vi "user process.vi"(8 "error in":errorcluster, 10 "ExampleStateMachine runtime in":refnum<class "ExampleStateMachine runtime.lvclass">, 11 "Parameters to process":T3) -> (0 "error out":errorcluster, 2 "ExampleStateMachine runtime out":refnum<class "ExampleStateMachine runtime.lvclass">, 3 "Results from processing":T2)   [LabVIEW 2017, in "ExampleStateMachine runtime.lvclass"]
uses:
  ExampleStateMachine runtime.lvclass
  parameter user data.ctl
  result user data.ctl
  Utilities/StateMachine.ctl
  Utilities/Controlword_Commands.ctl
  CommandCluster.ctl
  Utilities/WordManipulationLibrary.lvlib
panel:
  out "Status":T1
  out "Results":dbl[](array[numeric])
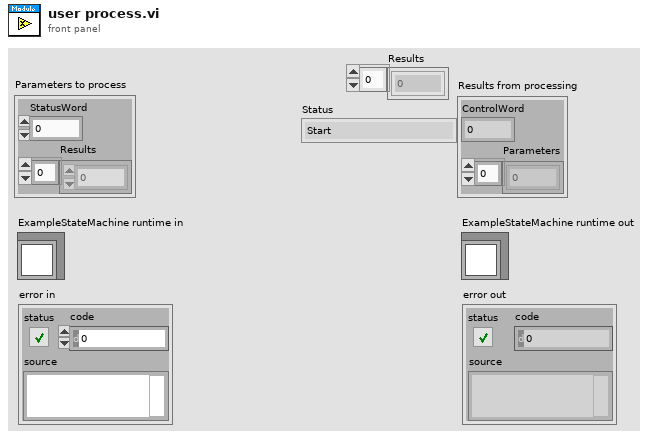
[diagram p1: front panel]
types:
  T1 = typedef "WordManipulationLibrary.lvlib/StateMachine.ctl" = enum16{"Start", "Not Ready to Switch On", "Switch On Disabled", "Ready to Switch On", "Switched On", "Operation enable", "Quick Stop Active", "Fault Reaction Active", "Fault"}
  T2 = typedef "ExampleStateMachine runtime.lvclass/result user data.ctl" = cluster{"ControlWord":u16, "Parameters":dbl[]}
  T3 = typedef "ExampleStateMachine runtime.lvclass/parameter user data.ctl" = cluster{"StatusWord":u16, "Results":dbl[]}
  T4 = typedef "WordManipulationLibrary.lvlib/Controlword_Commands.ctl" = enum16{"Shutdown", "Switch On", "Disable Voltage", "Quick Stop", "Disable Op", "Enable Op", "Fault Reset", "Error"}
  T5 = enum16{"Shutdown", "Switch On", "Disable Voltage", "Quick Stop", "Disable Op", "Enable Op", "Fault Reset", "Error"}
  T6 = typedef "CommandCluster.ctl" = cluster{"Modes":enum16{"Reserved", "Profile Position Mode", "Velocity Mode", "Profile Velocity Mode", "Profile Torque Mode", "Reserved 2", "Reference Mode", "Interpolated Position Mode", "Skip"}, "Parameters_PositionProfile":dbl[]}
  T7 = enum16{"Reserved", "Profile Position Mode", "Velocity Mode", "Profile Velocity Mode", "Profile Torque Mode", "Reserved 2", "Reference Mode", "Interpolated Position Mode", "Skip"}
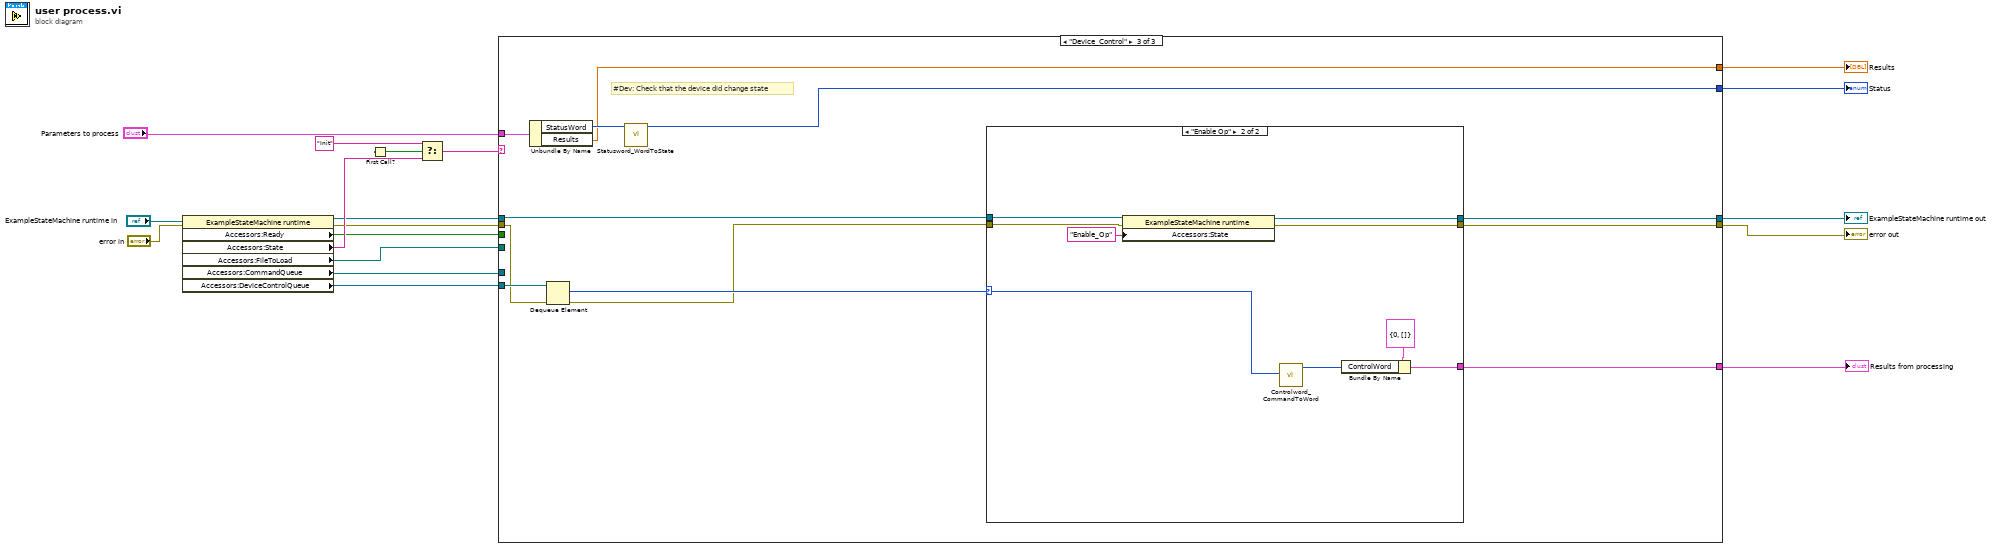
[diagram p0: block diagram]
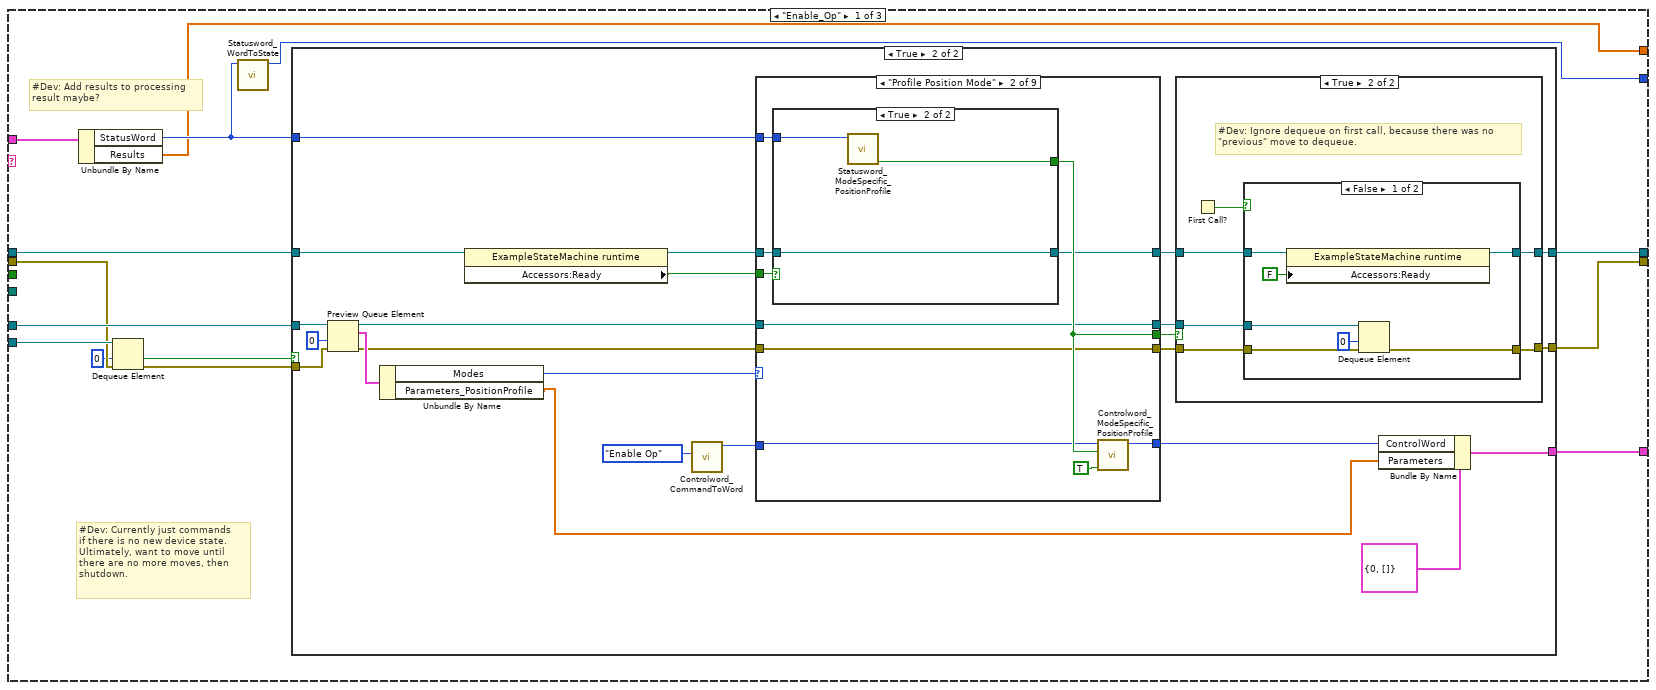
[diagram p2: hidden frame]
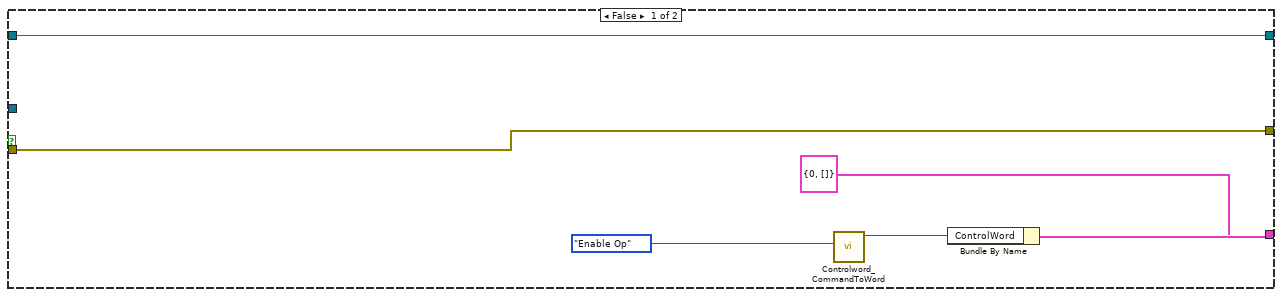
[diagram p3: hidden frame]
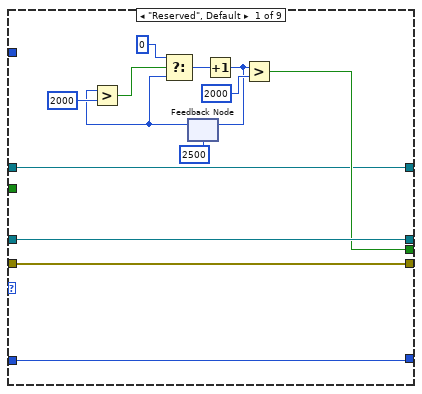
[diagram p6: hidden frame]
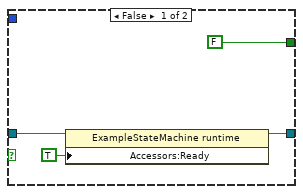
[diagram p7: hidden frame]
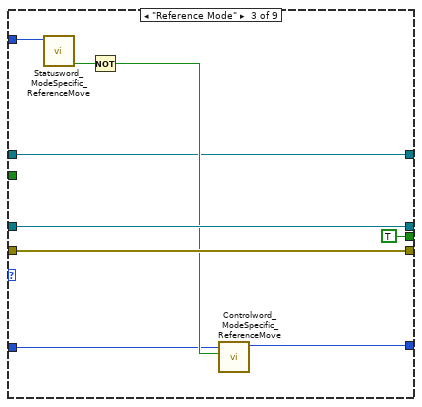
[diagram p8: hidden frame]
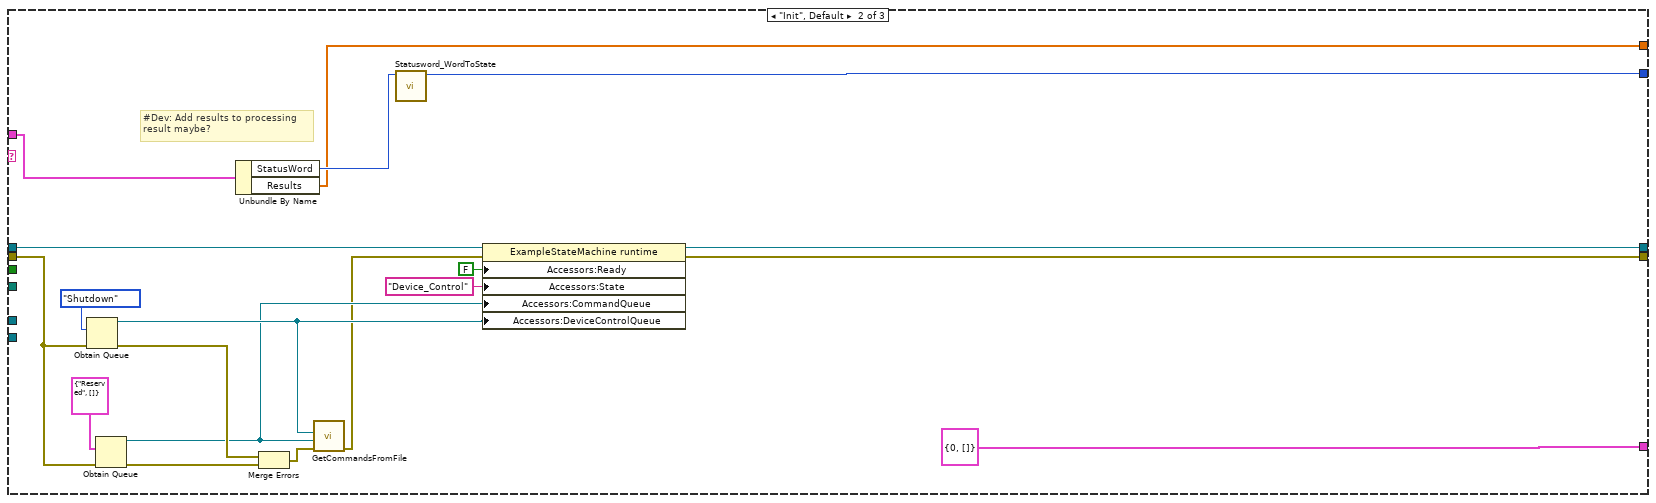
[diagram p15: hidden frame]
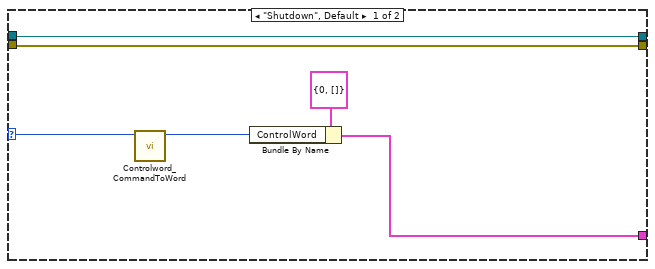
[diagram p16: hidden frame]
diagram:
  n1 = property class="ExampleStateMachine runtime"(reference="ExampleStateMachine runtime in", error in="error in") -> (reference out=w9:refnum<class "ExampleStateMachine runtime.lvclass">, error out=w7:errorcluster, "Accessors:Ready"=w5:bool, "Accessors:State"=w16:string, "Accessors:FileToLoad"=w10:path, "Accessors:CommandQueue"=w3:refnum<queue>, "Accessors:DeviceControlQueue"=w4:refnum<queue>)
  n2 = First Call?() -> (First Call?: T/F=w18:bool)
  n3 = Select(t="Init" ("f"), s=w18, f=w16) -> (s? t:f=w13:string)
  n4 = case shown="\"Device_Control\"" w13 {
    tunnel: "Parameters to process" -> [w26 w144 w170]
    tunnel: [w27 T2 {"ControlWord"=0, "Parameters"=[]} ("Results from processing") w172] -> w11
    tunnel: w10 -> [_ _ _]
    tunnel: w9 -> [w31 w159 w171]
    tunnel: [w24 w158 w166] -> w8
    tunnel: w7 -> [w29 w155 w165]
    tunnel: [w25 w157 w163] -> w6
    tunnel: w5 -> [_ _ _]
    tunnel: w4 -> [w32 _ w168]
    tunnel: w3 -> [w30 _ _]
    tunnel: [w22 w143 w162] -> w2
    tunnel: [w21 w142 w161] -> w1
    frame "Enable_Op" {
      # "#Dev: Add results to processing\nresult maybe?"
      # "#Dev: Currently just commands\nif there is no new device state.\nUltimately, want to move until\nthere are no more moves, then\nshutdown."
      n5 = Unbundle By Name(w26) -> ("StatusWord"=w23:u16, "Results"=w21:dbl[])
      n6 = Dequeue Element(queue=w32, timeout in ms (-1)=0, error in (no error)=w29) -> (timed out?=w19:bool, error out=w28:errorcluster)  [unwired: 2 out]
      n7 = call "Statusword_WordToState.vi"("Data_In"=w23) -> ("Status"=w22:T1)  [unwired: 10 in]
      n8 = case shown="True" w19 {
        tunnel: w31 -> [w38 w46]
        tunnel: w30 -> [_ w57]
        tunnel: w28 -> [w37 w58]
        tunnel: [w35 w59] -> w27
        tunnel: w23 -> [_ w55]
        tunnel: [w37 w47] -> w25
        tunnel: [w38 w40] -> w24
        frame False {
          n9 = call "Controlword_CommandToWord.vi"("Device Control Command"=Controlword_Commands."Enable Op") -> ("ControlWord Out"=w33:u16)  [unwired: 10 in]
          n10 = Bundle By Name(cluster=T2 {"ControlWord"=0, "Parameters"=[]} ("Results from processing"), "ControlWord"=w33) -> (w35:T2)
        }
        frame True {
          n11 = Preview Queue Element(queue=w57, timeout in ms (-1)=0, error in (no error)=w58) -> (queue out=w54:refnum<queue>, element=w56:T6, error out=w53:errorcluster)  [unwired: 1 out]
          n12 = Unbundle By Name(w56) -> ("Modes"=w50:T7, "Parameters_PositionProfile"=w42:dbl[])
          n13 = property class="ExampleStateMachine runtime"(reference=w46) -> (reference out=w44:refnum<class "ExampleStateMachine runtime.lvclass">, "Accessors:Ready"=w45:bool)  [unwired: 1 in, 1 out]
          n14 = call "Controlword_CommandToWord.vi"("Device Control Command"=Controlword_Commands."Enable Op") -> ("ControlWord Out"=w48:u16)  [unwired: 10 in]
          n15 = case shown="\"Profile Position Mode\"" w50 {
            tunnel: [w89 w100 w112 w119 w123 w127 w131 w135 w139] -> w61
            tunnel: w55 -> [_ w99 w114 _ _ _ _ _ _]
            tunnel: w54 -> [w91 w95 w117 w121 w125 w129 w133 w137 w141]
            tunnel: w53 -> [w90 w94 w116 w120 w124 w128 w132 w136 w140]
            tunnel: [w91 w95 w117 w121 w125 w129 w133 w137 w141] -> w52
            tunnel: [w90 w94 w116 w120 w124 w128 w132 w136 w140] -> w51
            tunnel: w48 -> [w89 w93 w111 w119 w123 w127 w131 w135 w139]
            tunnel: w45 -> [_ w98 _ _ _ _ _ _ _]
            tunnel: w44 -> [w80 w97 w109 w118 w122 w126 w130 w134 w138]
            tunnel: [w85 w96 TRUE ("Set Point Reached?") _ _ _ _ _ _] -> w43
            tunnel: [w80 w92 w109 w118 w122 w126 w130 w134 w138] -> w41
            frame "Reserved", Default {
              n16 = feedback #1(2500) -> (w81:i32)
              n17 = Greater?(x=w81, y=2000) -> (0:w82:bool)
              n18 = Select(t=0, s=w82, f=w81) -> (s? t:f=w86:i32)
              n19 = Increment(x=w86) -> (x+1=w84:i32)
              n20 = feedback-in #1(w84) -> ()
              n21 = Greater?(x=w84, y=2000) -> (0:w85:bool)
            }
            frame "Profile Position Mode" {
              n22 = case shown="True" w98 {
                tunnel: w99 -> [_ w108]
                tunnel: [FALSE ("Set Point Reached?") w107] -> w96
                tunnel: w97 -> [w104 w106]
                tunnel: [w102 w106] -> w92
                frame False {
                  n23 = property class="ExampleStateMachine runtime"(reference=w104, "Accessors:Ready"=TRUE ("Ready")) -> (reference out=w102:refnum<class "ExampleStateMachine runtime.lvclass">)  [unwired: 1 in, 1 out]
                }
                frame True {
                  n24 = call "Statusword_ModeSpecific_PositionProfile.vi"("StatusWord In"=w108) -> ("Set Point Reached?"=w107:bool)  [unwired: 7 in, 3 out]
                }
              }
              n25 = call "Controlword_ModeSpecific_PositionProfile.vi"("Relative?"=TRUE ("Absolute?"), "New Setpoint?"=w96, "ControlWord In"=w93) -> ("ControlWord Out"=w100:u16)  [unwired: 8 in]
            }
            frame "Reference Mode" {
              n26 = call "Statusword_ModeSpecific_ReferenceMove.vi"("StatusWord In"=w114) -> ("Set Point Reached?"=w115:bool)  [unwired: 9 in, 1 out]
              n27 = Not(x=w115) -> (.not. x?=w113:bool)
              n28 = call "Controlword_ModeSpecific_ReferenceMove.vi"("Operation Start"=w113, "ControlWord In"=w111) -> ("ControlWord Out"=w112:u16)  [unwired: 9 in]
            }
            frame "Velocity Mode" {
            }
            frame "Profile Velocity Mode" {
            }
            frame "Profile Torque Mode" {
            }
            frame "Reserved 2" {
            }
            frame "Interpolated Position Mode" {
            }
            frame "Skip" {
            }
          }
          n29 = case shown="True" w43 {
            tunnel: w52 -> [_ w67]
            tunnel: w51 -> [w63 w69]
            tunnel: [w63 w68] -> w47
            tunnel: w41 -> [w62 w66]
            tunnel: [w62 w65] -> w40
            frame False {
            }
            frame True {
              # "#Dev: Ignore dequeue on first call, because there was no \n\"previous\" move to dequeue."
              n30 = First Call?() -> (First Call?: T/F=w64:bool)
              n31 = case shown="False" w64 {
                tunnel: w69 -> [w76 w77]
                tunnel: [w75 w77] -> w68
                tunnel: w67 -> [w74 _]
                tunnel: w66 -> [w73 w78]
                tunnel: [w72 w78] -> w65
                frame False {
                  n32 = property class="ExampleStateMachine runtime"(reference=w73, "Accessors:Ready"=FALSE ("Ready")) -> (reference out=w72:refnum<class "ExampleStateMachine runtime.lvclass">)  [unwired: 1 in, 1 out]
                  n33 = Dequeue Element(queue=w74, timeout in ms (-1)=0, error in (no error)=w76) -> (error out=w75:errorcluster)  [unwired: 3 out]
                }
                frame True {
                }
              }
            }
          }
          n34 = Bundle By Name(cluster=T2 {"ControlWord"=0, "Parameters"=[]} ("Results from processing"), "ControlWord"=w61, "Parameters"=w42) -> (w59:T2)
        }
      }
    }
    frame "Init", Default {
      # "#Dev: Add results to processing\nresult maybe?"
      n35 = Obtain Queue(element data type=T5."Shutdown" ("Device Control Command"), error in (no error)=w155) -> (queue out=w148:refnum<queue>, error out=w150:errorcluster)  [unwired: 3 in, 1 out]
      n36 = Obtain Queue(element data type=T6 {"Modes"=enum."Reserved", "Parameters_PositionProfile"=[]}, error in (no error)=w155) -> (queue out=w147:refnum<queue>, error out=w151:errorcluster)  [unwired: 3 in, 1 out]
      n37 = Unbundle By Name(w144) -> ("StatusWord"=w145:u16, "Results"=w142:dbl[])
      n38 = Merge Errors(w150, w151) -> (w149:errorcluster)
      n39 = call "GetCommandsFromFile.vi"("error in"=w149, "CommandQueue"=w147, "DeviceControlQueue"=w148) -> ("error out"=w146:errorcluster)  [unwired: 8 in]
      n40 = call "Statusword_WordToState.vi"("Data_In"=w145) -> ("Status"=w143:T1)  [unwired: 10 in]
      n41 = property class="ExampleStateMachine runtime"(reference=w159, error in=w146, "Accessors:Ready"=FALSE ("Running"), "Accessors:State"="Device_Control" ("State"), "Accessors:CommandQueue"=w147, "Accessors:DeviceControlQueue"=w148) -> (reference out=w158:refnum<class "ExampleStateMachine runtime.lvclass">, error out=w157:errorcluster)
    }
    frame "Device_Control" {
      # "#Dev: Check that the device did change state"
      n42 = Unbundle By Name(w170) -> ("StatusWord"=w169:u16, "Results"=w161:dbl[])
      n43 = Dequeue Element(queue=w168, error in (no error)=w165) -> (element=w167:T5, error out=w164:errorcluster)  [unwired: 1 in, 2 out]
      n44 = call "Statusword_WordToState.vi"("Data_In"=w169) -> ("Status"=w162:T1)  [unwired: 10 in]
      n45 = case shown="\"Enable Op\"" w167 {
        selector: w167 -> [w175 w179]
        tunnel: [w176 w180] -> w172
        tunnel: w171 -> [w174 w187]
        tunnel: [w174 w186] -> w166
        tunnel: w164 -> [w173 w184]
        tunnel: [w173 w183] -> w163
        frame "Shutdown", Default {
          n46 = call "Controlword_CommandToWord.vi"("ControlWord In"=w175) -> ("ControlWord Out"=w177:u16)  [unwired: 10 in]
          n47 = Bundle By Name(cluster=T2 {"ControlWord"=0, "Parameters"=[]} ("Results from processing"), "ControlWord"=w177) -> (w176:T2)
        }
        frame "Enable Op" {
          n48 = property class="ExampleStateMachine runtime"(reference=w187, error in=w184, "Accessors:State"="Enable_Op" ("State")) -> (reference out=w186:refnum<class "ExampleStateMachine runtime.lvclass">, error out=w183:errorcluster)
          n49 = call "Controlword_CommandToWord.vi"("Device Control Command"=w179) -> ("ControlWord Out"=w182:u16)  [unwired: 10 in]
          n50 = Bundle By Name(cluster=T2 {"ControlWord"=0, "Parameters"=[]} ("Results from processing"), "ControlWord"=w182) -> (w180:T2)
        }
      }
    }
  }
  "error out" <- w6
  "Results from processing" <- w11
  "ExampleStateMachine runtime out" <- w8
  "Status" <- w2
  "Results" <- w1
